vi "Tests - Test UTF-8 validation.vi"() -> ()   [LabVIEW 2019, in "KoRE-MQTT.lvlib"]
doc: "Copyright (c) 2025 KoRElibs.com\nSPDX-License-Identifier: EUPL-1.2\n\nThis VI is licensed under the European Union Public License (EUPL) Version 1.2. You may use this VI unmodified in proprietary works. If you distribute a modified version of this file, the modified file must be released under the EUPL-1.2. Full license: https://joinup.ec.europa.eu/asset/eupl/eupl/1.2/"
uses:
  KoRE-MQTT.lvlib
panel:
  out "Failed":string[](array[string])
  out "Passed":string[](array[string])
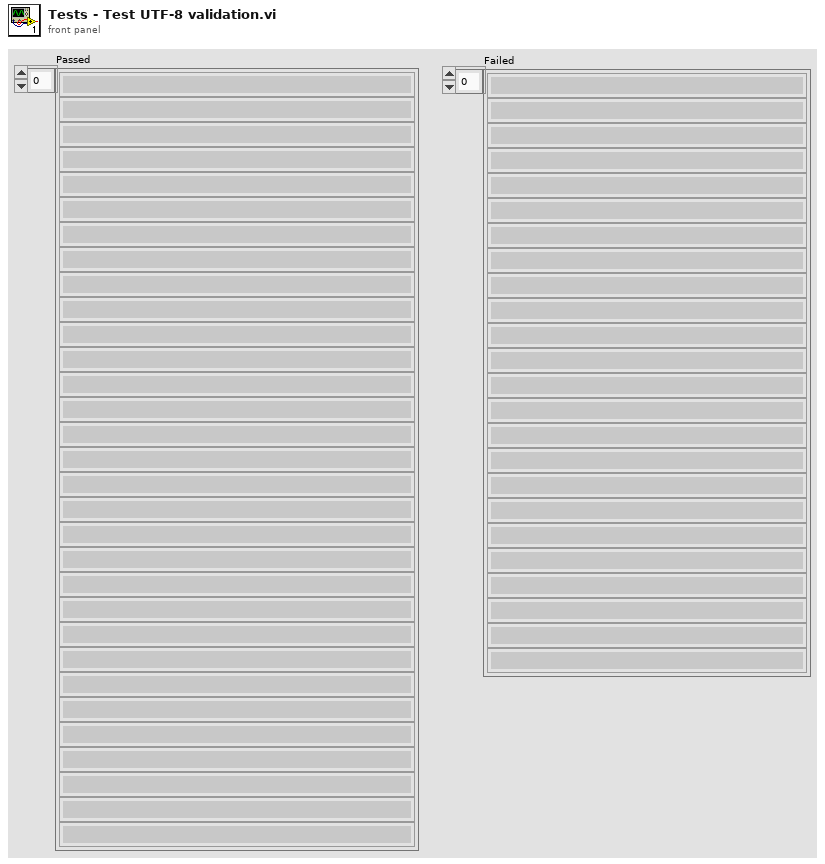
[diagram p1: front panel]
types:
  T1 = cluster{"description":string, "valid":bool, "bytes":u8[]}[]
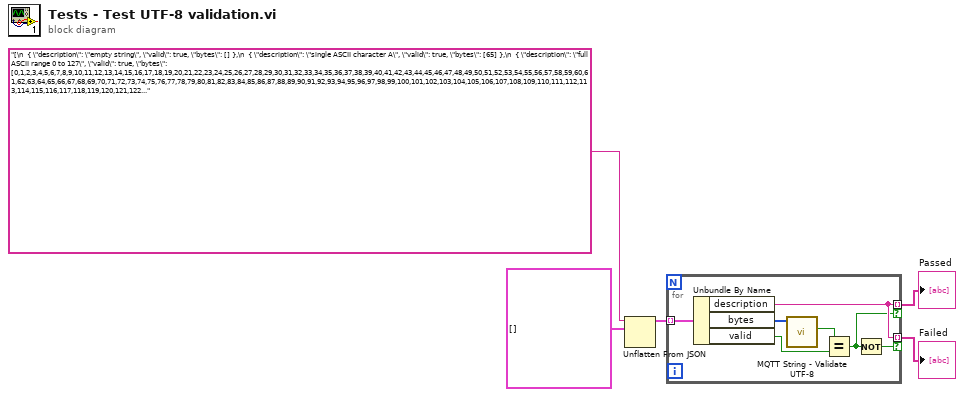
[diagram p0: block diagram]
diagram:
  n1 = Unflatten From JSON(JSON string="[\n  { \"description\": \"empty string\", \"valid\": true, \"bytes\": [] },\n  { \"description\": \"single ASCII character A\", \"valid\": true, \"bytes\": [65] },\n  { \"description\": \"full ASCII range 0 to 127\", \"valid\": true, \"bytes\": [0,1,2,3,4,5,6,7,8,9,10,11,12,13,14,15,16,17,18,19,20,21,22,23,24,25,26,27,28,29,30,31,32,33,34,35,36,37,38,39,40,41,42,43,44,45,46,47,48,49,50,51,52,53,54,55,56,57,58,59,60,61,62,63,64,65,66,67,68,69,70,71,72,73,74,75,76,77,78,79,80,81,82,83,84,85,86,87,88,89,90,91,92,93,94,95,96,97,98,99,100,101,102,103,104,105,106,107,108,109,110,111,112,113,114,115,116,117,118,119,120,121,122,123,124,125,126,127] },\n\n  { \"description\": \"valid two byte sequence for cent sign\", \"valid\": true, \"bytes\": [194,162] },\n  { \"description\": \"valid two byte sequence for latin small letter y with diaeresis\", \"valid\": true, \"bytes\": [195,191] },\n  { \"description\": \"overlong encoding of slash (invalid)\", \"valid\": false, \"bytes\": [192,175] },\n  { \"description\": \"overlong encoding of null (invalid)\", \"valid\": false, \"bytes\": [192,128] },\n  { \"description\": \"truncated two byte start (invalid)\", \"valid\": false, \"bytes\": [194] },\n  { \"description\": \"invalid start byte C0 (reserved, invalid)\", \"valid\": false, \"bytes\": [192,128] },\n  { \"description\": \"invalid start byte C1 (reserved, invalid)\", \"valid\": false, \"bytes\": [193,130] },\n\n  { \"description\": \"valid three byte sequence for euro sign\", \"valid\": true, \"bytes\": [226,130,172] },\n  { \"description\": \"valid three byte sequence for Hangul syllable GA\", \"valid\": true, \"bytes\": [234,176,128] },\n  { \"description\": \"overlong encoding of at sign (invalid)\", \"valid\": false, \"bytes\": [224,128,128] },\n  { \"description\": \"truncated three byte start (invalid)\", \"valid\": false, \"bytes\": [226,130] },\n  { \"description\": \"invalid three byte start with illegal second continuation (invalid)\", \"valid\": false, \"bytes\": [226,255,128] },\n  { \"description\": \"invalid three byte start with illegal third continuation (invalid)\", \"valid\": false, \"bytes\": [226,130,0] },\n  { \"description\": \"surrogate high (U+D800) invalid\", \"valid\": false, \"bytes\": [237,160,128] },\n  { \"description\": \"surrogate low (U+DC00) invalid\", \"valid\": false, \"bytes\": [237,176,128] },\n\n  { \"description\": \"valid four byte sequence for grinning face emoji\", \"valid\": true, \"bytes\": [240,159,152,128] },\n  { \"description\": \"valid four byte sequence for Gothic letter\", \"valid\": true, \"bytes\": [240,144,141,136] },\n  { \"description\": \"overlong encoding of null in four bytes (invalid)\", \"valid\": false, \"bytes\": [240,128,128,128] },\n  { \"description\": \"code point greater than U+10FFFF (invalid)\", \"valid\": false, \"bytes\": [244,144,128,128] },\n  { \"description\": \"truncated four byte start (invalid)\", \"valid\": false, \"bytes\": [240,159,152] },\n  { \"description\": \"invalid four byte start followed by illegal start byte 0xFF (invalid)\", \"valid\": false, \"bytes\": [240,159,152,255] },\n\n  { \"description\": \"single continuation byte (invalid)\", \"valid\": false, \"bytes\": [128] },\n  { \"description\": \"two continuation bytes (invalid)\", \"valid\": false, \"bytes\": [128,128] },\n\n  { \"description\": \"ASCII followed by valid two, three and four byte sequences\", \"valid\": true, \"bytes\": [65,194,162,226,130,172,240,159,152,128] },\n  { \"description\": \"ASCII followed by truncated two byte start (invalid)\", \"valid\": false, \"bytes\": [65,194] },\n  { \"description\": \"ASCII followed by truncated three byte start (invalid)\", \"valid\": false, \"bytes\": [65,226,130] },\n  { \"description\": \"ASCII followed by truncated four byte start (invalid)\", \"valid\": false, \"bytes\": [65,240,159,152] },\n  {  \"description\": \"UTF-8 BOM (0xEF 0xBB 0xBF) must be accepted as U+FEFF\", \"valid\": true, \"bytes\": [239, 187, 191] }\n]\n", type and defaults=T1 []) -> (value=w3:T1)  [unwired: 5 in, 1 out]
  n2 = for {
    tunnel: w3 -> [w12] mode=indexing
    tunnel: [w9] -> w2 mode=indexing if=w8
    tunnel: [w9] -> w1 mode=indexing if=w7
    n3 = Unbundle By Name(w12) -> ("description"=w9:string, "bytes"=w11:u8[], "valid"=w10:bool)
    n4 = call "MQTT String - Validate UTF-8.vi"("UTF-8 Data"=w11) -> ("Valid"=w6:bool)  [unwired: 10 in]
    n5 = Equal?(x=w6, y=w10) -> (x = y?=w8:bool)
    n6 = Not(x=w8) -> (.not. x?=w7:bool)
  }
  "Passed" <- w2
  "Failed" <- w1
